vi "RFH-verify-LibreVNA_conversion.vi"(5 "Conversion Folder":path, 7 "Excel File Folder":path, 8 "error in (no error)":errorcluster, 9 "Max Frequency (6G)":dbl=6000000000.0, 10 "Min Frequency  (0.3G)":dbl=300000000.0) -> (0 "error out":errorcluster, 3 "All Good?":bool)   [LabVIEW 2020, in "RFH-Reflection_File_Handler.lvlib"]
doc: "Verifies converted LibreVNA files against their source data, value by value and in the min and max frequency range. Returns whether all are good."
uses:
  RFH-Reflection_File_Handler.lvlib
  RFH-common_data_format_element.ctl
panel:
  out "Range Good?":bool
  out "Values Good?":bool
  out "All Files in Dir":path[](array[path])
  out "value 4":T1
  out "value 3":T1
  out "value 2":T1
  out "value":T1
  out "Array":bool[](array[boolean])
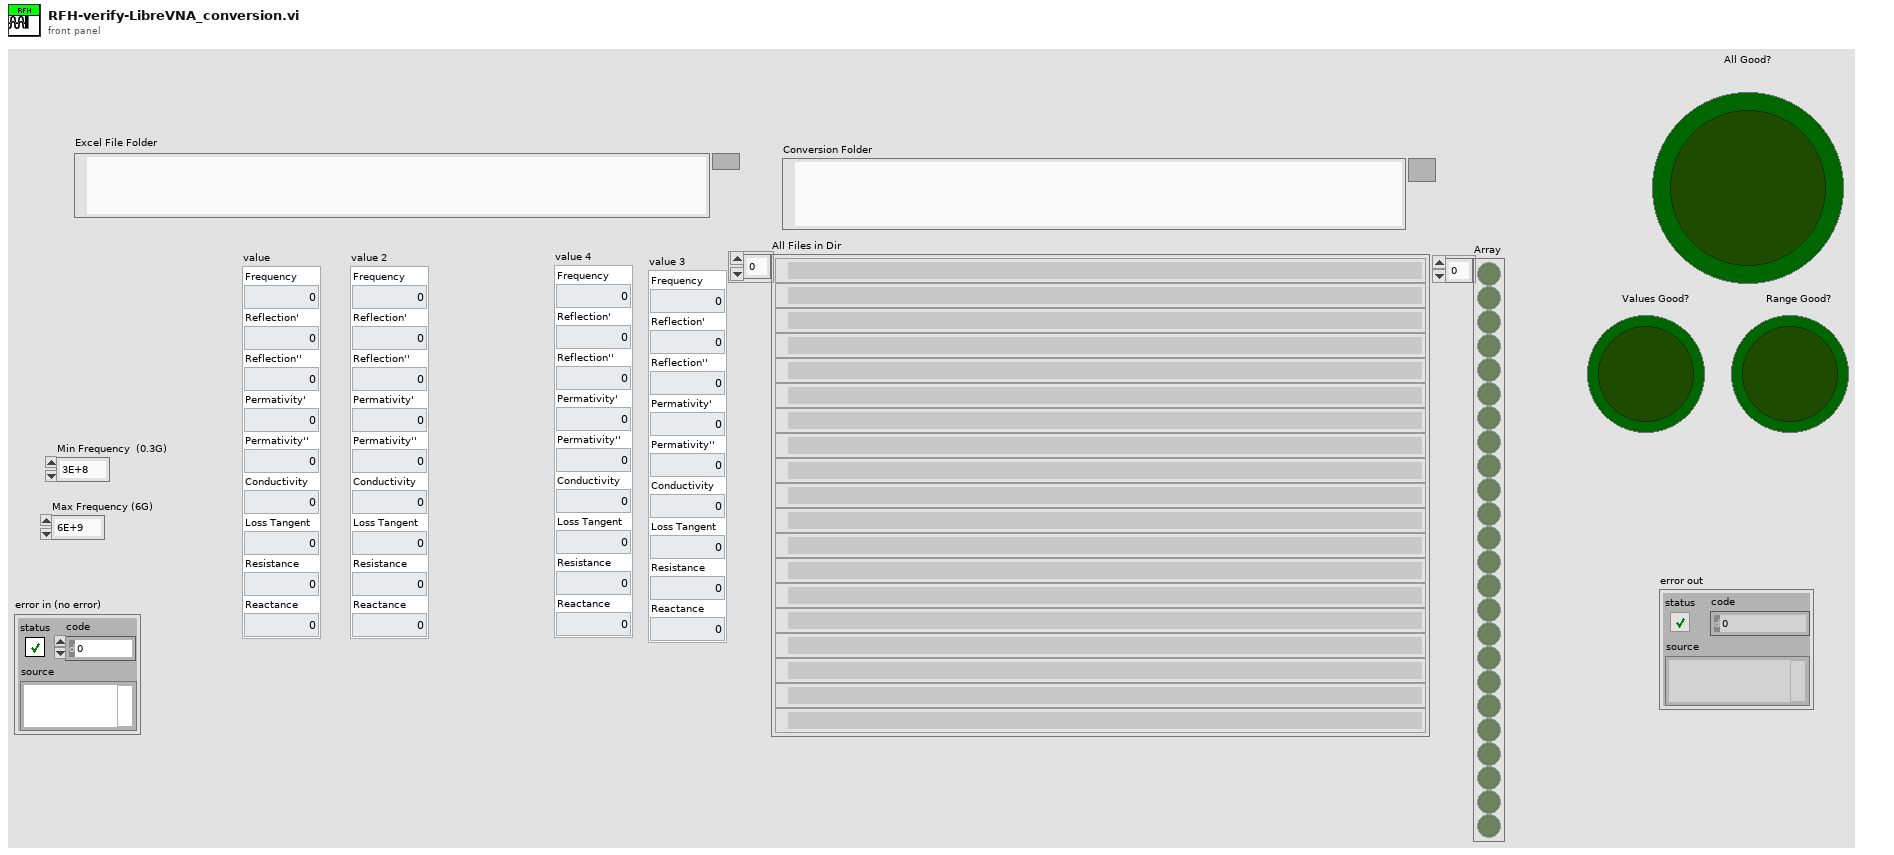
[diagram p1: front panel]
types:
  T1 = typedef "RFH-Reflection_File_Handler.lvlib/RFH-common_data_format_element.ctl" = cluster{"Frequency":dbl, "Reflection'":dbl, "Reflection''":dbl, "Permativity'":dbl, "Permativity''":dbl, "Conductivity":dbl, "Loss Tangent":dbl, "Resistance":dbl, "Reactance":dbl}
  T2 = typedef "RFH-Reflection_File_Handler.lvlib/RFH-common_data_format.ctl" = cluster{"Frequency":dbl[], "Reflection'":dbl[], "Reflection''":dbl[], "Permativity'":dbl[], "Permativity''":dbl[], "Conductivity":dbl[], "Loss Tangent":dbl[], "Resistance":dbl[], "Reactance":dbl[]}
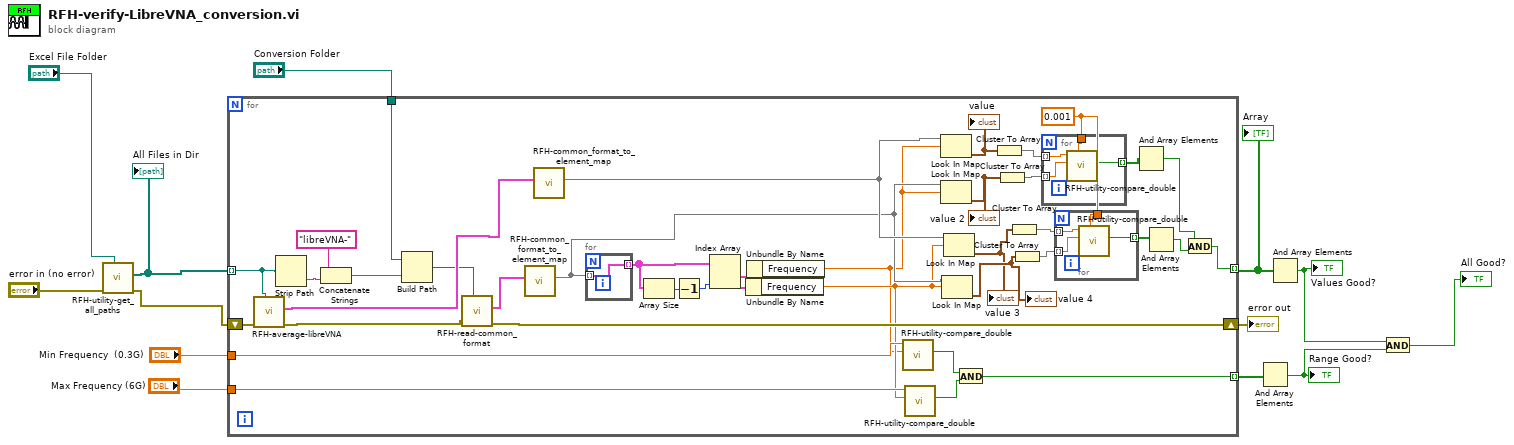
[diagram p0: block diagram]
diagram:
  n1 = call "RFH-utility-get_all_paths.vi"("Folder Path"="Excel File Folder", "error in (no error)"="error in (no error)") -> ("error out"=w9:errorcluster, "All Folders"=w8:path[])  [unwired: 6 in, 2 out]
  "All Files in Dir" <- w8
  n2 = for {
    tunnel: w8 -> [w24] mode=indexing
    tunnel: "Conversion Folder" -> [w22]
    shift-right: [w52] -> w13
    shift-left: w9 -> [w29]
    tunnel: [w43] -> w11 mode=indexing
    tunnel: "Min Frequency  (0.3G)" -> [w20]
    tunnel: "Max Frequency (6G)" -> [w19]
    tunnel: [w14] -> w5 mode=indexing
    w30 = 0.001 ("% tolerance (0.1)")
    n3 = call "RFH-average-libreVNA.vi"("Source Folder"=w24, "error in (no error)"=w29) -> ("error out"=w21:errorcluster, "Common Format"=w28:T2)  [unwired: 8 in]
    n4 = Strip Path(path=w24) -> (name=w25:string)  [unwired: 1 out]
    n5 = Concatenate Strings("libreVNA-" ("string"), w25) -> (w27:string)
    n6 = Build Path(base path=w22, name or relative path=w27) -> (appended path=w23:path)
    n7 = call "RFH-read-common_format.vi"("file path (dialog if empty)"=w23, "error in"=w21) -> ("error out"=w52:errorcluster, "Common Format"=w51:T2)  [unwired: 8 in]
    n8 = call "RFH-common_format_to_element_map.vi"("Common Format"=w51) -> ("Element map"=w44:map{dbl, T1})  [unwired: 10 in]
    n9 = call "RFH-common_format_to_element_map.vi"("Common Format"=w28) -> ("Element map"=w45:map{dbl, T1})  [unwired: 10 in]
    n10 = for {
      tunnel: w44 -> [w61] mode=indexing
      tunnel: [w61] -> w48 mode=indexing
    }
    n11 = Array Size(array=w48) -> (size(s)=w49:i32)
    n12 = Decrement(x=w49) -> (x-1=w50:i32)
    n13 = Index Array(array=w48, index #2=w50) -> (element #1=w46:cluster{"Frequency":dbl, "Common Format":T1}, element #2=w47:cluster{"Frequency":dbl, "Common Format":T1})  [unwired: 1 in]
    n14 = Unbundle By Name(w47) -> ("Frequency"=w18:dbl)
    n15 = Unbundle By Name(w46) -> ("Frequency"=w17:dbl)
    n16 = call "RFH-utility-compare_double.vi"("New"=w17, "original"=w20) -> ("In Range?"=w16:bool)  [unwired: 9 in]
    n17 = call "RFH-utility-compare_double.vi"("New"=w18, "original"=w19) -> ("In Range?"=w15:bool)  [unwired: 9 in]
    n18 = Look In Map(map=w45, key=w17) -> (value=w42:T1)  [unwired: 1 in, 1 out]
    "value" <- w42
    n19 = Look In Map(map=w44, key=w17) -> (value=w41:T1)  [unwired: 1 in, 1 out]
    "value 2" <- w41
    n20 = Look In Map(map=w44, key=w18) -> (value=w36:T1)  [unwired: 1 in, 1 out]
    "value 4" <- w36
    n21 = Look In Map(map=w45, key=w18) -> (value=w35:T1)  [unwired: 1 in, 1 out]
    "value 3" <- w35
    n22 = And(x=w16, y=w15) -> (x .and. y?=w14:bool)
    n23 = Cluster To Array(cluster=w42) -> (array=w40:dbl[])
    n24 = Cluster To Array(cluster=w41) -> (array=w39:dbl[])
    n25 = Cluster To Array(cluster=w35) -> (array=w37:dbl[])
    n26 = Cluster To Array(cluster=w36) -> (array=w38:dbl[])
    n27 = for {
      tunnel: w40 -> [w60] mode=indexing
      tunnel: w39 -> [w59] mode=indexing
      tunnel: [w58] -> w31 mode=indexing
      tunnel: w30 -> [w57]
      n28 = call "RFH-utility-compare_double.vi"("% tolerance (0.1)"=w57, "New"=w59, "original"=w60) -> ("In Range?"=w58:bool)  [unwired: 8 in]
    }
    n29 = for {
      tunnel: w37 -> [w56] mode=indexing
      tunnel: w38 -> [w55] mode=indexing
      tunnel: [w54] -> w33 mode=indexing
      tunnel: w30 -> [w53]
      n30 = call "RFH-utility-compare_double.vi"("% tolerance (0.1)"=w53, "New"=w55, "original"=w56) -> ("In Range?"=w54:bool)  [unwired: 8 in]
    }
    n31 = And Array Elements(Boolean array=w31) -> (logical AND=w32:bool)
    n32 = And Array Elements(Boolean array=w33) -> (logical AND=w34:bool)
    n33 = And(x=w32, y=w34) -> (x .and. y?=w43:bool)
  }
  "error out" <- w13
  "Array" <- w11
  n34 = And Array Elements(Boolean array=w5) -> (logical AND=w4:bool)
  "Range Good?" <- w4
  n35 = And Array Elements(Boolean array=w11) -> (logical AND=w3:bool)
  "Values Good?" <- w3
  n36 = And(x=w3, y=w4) -> (x .and. y?=→"All Good?":bool)
